vi "writeVisaMaybe.vi"(4 "String to Write":string, 5 "error in":errorcluster, 6 "VISA resource name in":refnum<visa-resource-name>, 7 "VISA connected?":bool) -> (1 "error out":errorcluster, 2 "VISA resource name out":refnum<visa-resource-name>)   [LabVIEW 2025]
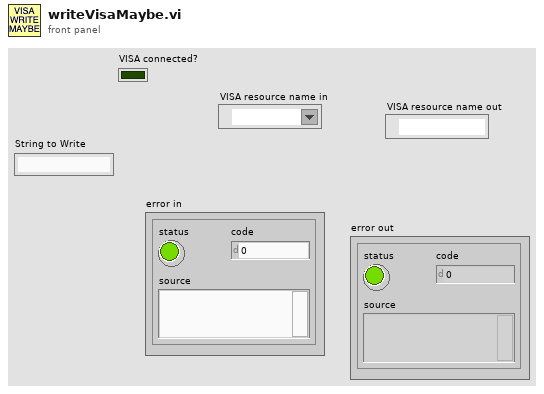
[diagram p1: front panel]
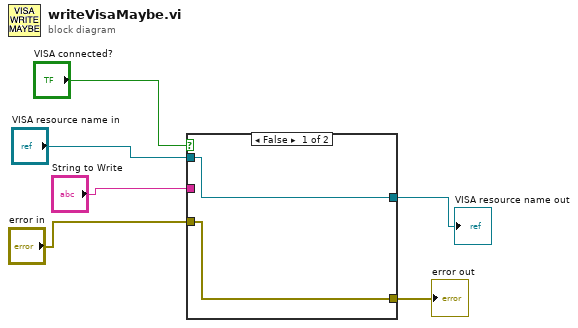
[diagram p0: block diagram]
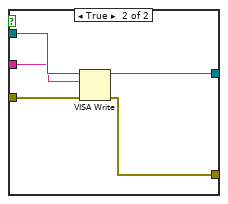
[diagram p2: hidden frame]
diagram:
  n1 = case shown="False" "VISA connected?" {
    tunnel: "VISA resource name in" -> [w8 w13]
    tunnel: "String to Write" -> [_ w12]
    tunnel: "error in" -> [w7 w11]
    tunnel: [w7 w10] -> w2
    tunnel: [w8 w9] -> w1
    frame False {
    }
    frame True {
      n2 = VISA Write(VISA resource name=w13, write buffer=w12, error in (no error)=w11) -> (VISA resource name out=w9:refnum<visa-resource-name>, error out=w10:errorcluster)  [unwired: 1 out]
    }
  }
  "error out" <- w2
  "VISA resource name out" <- w1
